vi "DAQ_Scale.vi"(0 "Raw Data (A)":dbl[][](array[numeric]), 5 "Channels":T1(array[cluster]), 11 "error in":errorcluster) -> (4 "Scaled Data":dbl[][](array[numeric]), 6 "Values":dbl[](array[numeric]), 15 "error out":errorcluster)   [LabVIEW 2026]
doc: "채널별 4~20 mA 선형 환산: y = Scale Min + (I - 4 mA) x (Scale Max - Scale Min) / 16 mA.\nValues = 채널별 평균(디지털 인디케이터 표시값)."
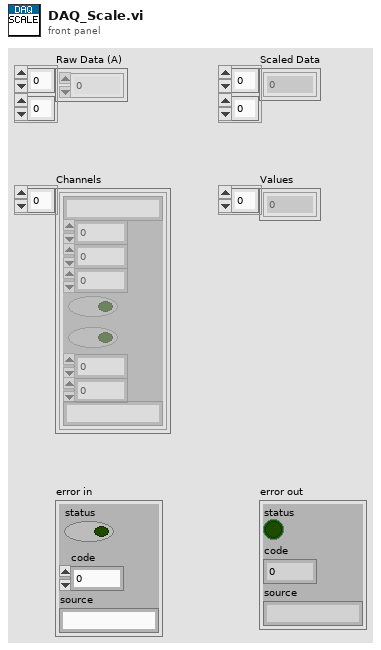
[diagram p1: front panel]
types:
  T1 = cluster{"Name":string, "Value":dbl, "High Limit":dbl, "Low Limit":dbl, "Save":bool, "Graph":bool, "Scale Min":dbl, "Scale Max":dbl, "Unit":string}[]
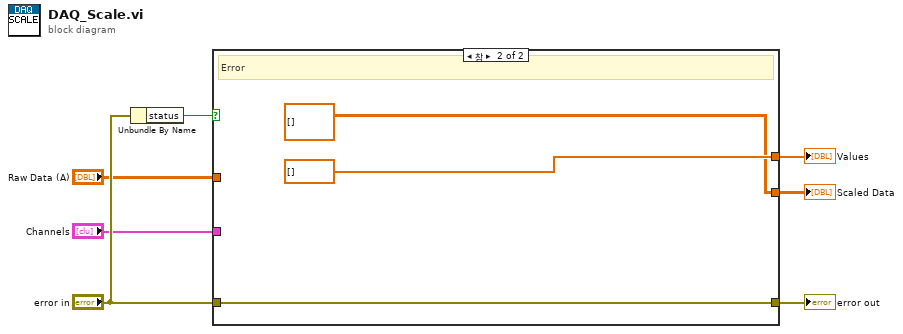
[diagram p0: block diagram]
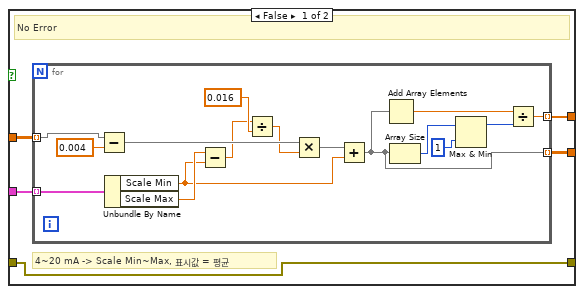
[diagram p2: hidden frame]
diagram:
  n1 = Unbundle By Name("error in") -> ("status"=w4:bool)
  n2 = case shown="참" w4 {
    tunnel: "Raw Data (A)" -> [w8 _]
    tunnel: "Channels" -> [w9 _]
    tunnel: "error in" -> [w10 w29]
    tunnel: [w10 w29] -> w7
    tunnel: [w11 dbl[][] []] -> w5
    tunnel: [w12 dbl[] []] -> w6
    frame False {
      # "4~20 mA -> Scale Min~Max, 표시값 = 평균"
      # "No Error"
      n3 = for {
        tunnel: w8 -> [w13] mode=indexing
        tunnel: w9 -> [w14] mode=indexing
        tunnel: [w23] -> w11 mode=indexing
        tunnel: [w28] -> w12 mode=indexing
        n4 = Subtract(x=w13, y=0.004) -> (x-y=w21:dbl[])
        n5 = Unbundle By Name(w14) -> ("Scale Min"=w15:dbl, "Scale Max"=w16:dbl)
        n6 = Subtract(x=w16, y=w15) -> (x-y=w17:dbl)
        n7 = Divide(x=w17, y=0.016) -> (x/y=w19:dbl)
        n8 = Multiply(x=w21, y=w19) -> (x*y=w22:dbl[])
        n9 = Add(x=w22, y=w15) -> (x+y=w23:dbl[])
        n10 = Add Array Elements(numeric array=w23) -> (sum=w25:dbl)
        n11 = Array Size(array=w23) -> (size(s)=w24:i32)
        n12 = Max & Min(x=w24, y=1) -> (max(x,y)=w27:i32)  [unwired: 1 out]
        n13 = Divide(x=w25, y=w27) -> (x/y=w28:dbl)
      }
    }
    frame True {
      # "Error"
    }
  }
  "Scaled Data" <- w5
  "Values" <- w6
  "error out" <- w7
